vi "HI_LO_SET_TYPE.vi"(8 "error out":errorcluster, 11 "Enum":T1) -> (0 "error out":errorcluster, 2 "LOW SET":string, 3 "HI SET":string)   [LabVIEW 2021]
uses:
  HI-POT_Driver/Hi-pot_Driver.ctl
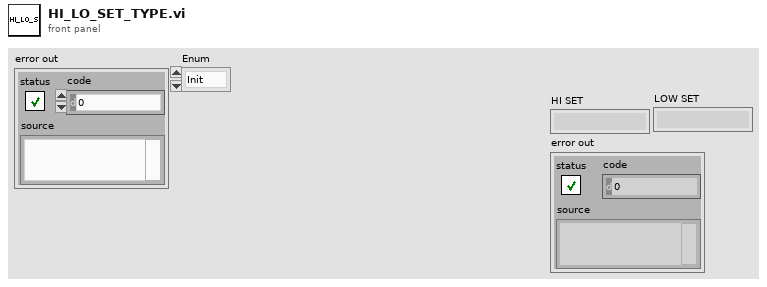
[diagram p1: front panel]
types:
  T1 = typedef "Hi-pot_Driver.ctl" = enum16{"Init ", "Interlock status", "Set UP DCW", "Set UP ACW", "Set UP IR", "Read", "Clear", "Close"}
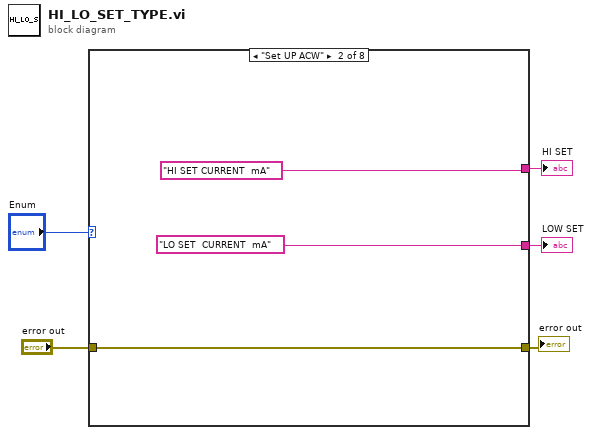
[diagram p0: block diagram]
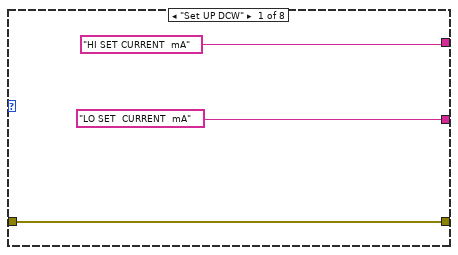
[diagram p2: hidden frame]
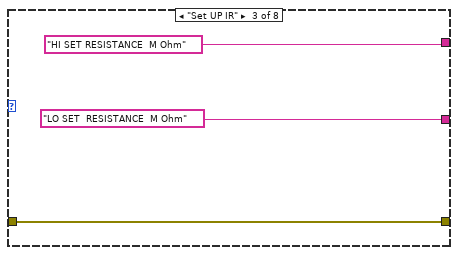
[diagram p3: hidden frame]
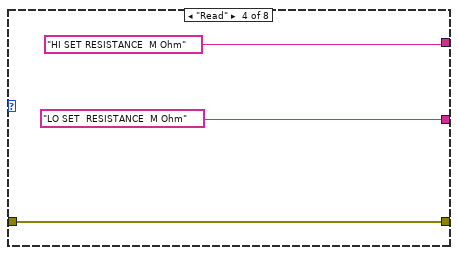
[diagram p4: hidden frame]
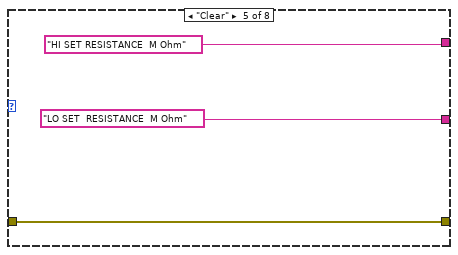
[diagram p5: hidden frame]
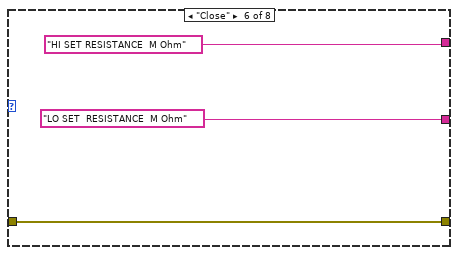
[diagram p6: hidden frame]
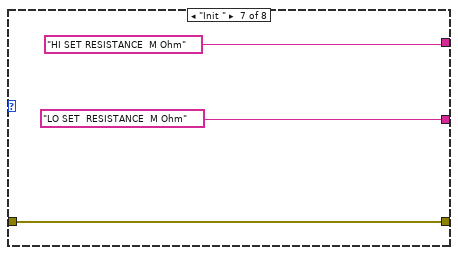
[diagram p7: hidden frame]
diagram:
  n1 = case shown="\"Set UP ACW\"" "Enum" {
    tunnel: ["HI SET CURRENT  mA" ("Expected 2") "HI SET CURRENT  mA" ("Expected 2") "HI SET RESISTANCE  M Ohm" ("Expected 2") "HI SET RESISTANCE  M Ohm" ("Expected 2") "HI SET RESISTANCE  M Ohm" ("Expected 2") "HI SET RESISTANCE  M Ohm" ("Expected 2") "HI SET RESISTANCE  M Ohm" ("Expected 2") _] -> w5
    tunnel: ["LO SET  CURRENT  mA" ("String Indicator 6") "LO SET  CURRENT  mA" ("String Indicator 6") "LO SET  RESISTANCE  M Ohm" ("String Indicator 6") "LO SET  RESISTANCE  M Ohm" ("String Indicator 6") "LO SET  RESISTANCE  M Ohm" ("String Indicator 6") "LO SET  RESISTANCE  M Ohm" ("String Indicator 6") "LO SET  RESISTANCE  M Ohm" ("String Indicator 6") _] -> w4
    tunnel: "error out" -> [w6 w9 w12 w15 w18 w21 w24 w27]
    tunnel: [w6 w9 w12 w15 w18 w21 w24 w27] -> w2
    frame "Set UP DCW" {
    }
    frame "Set UP ACW" {
    }
    frame "Set UP IR" {
    }
    frame "Read" {
    }
    frame "Clear" {
    }
    frame "Close" {
    }
    frame "Init " {
    }
    frame "Interlock status" {
    }
  }
  "HI SET" <- w5
  "LOW SET" <- w4
  "error out" <- w2
